vi "set FCC Part15c U-NII-1 Integration BE mode.vi"(8 "error in (no error)":errorcluster, 11 "Band Edge in":refnum<class "Band Edge.lvclass">) -> (0 "error out":errorcluster, 3 "Band Edge out":refnum<class "Band Edge.lvclass">)   [LabVIEW 2023, in "Spectrum Analyzer.lvlib" / "Band Edge.lvclass"]
uses:
  Band Edge.lvclass
  Band Edge.lvclass/Band Edge.ctl
  TYPE DEFINITION/TYPE RBW and VBW Select.ctl
  Spectrum Analyzer.lvlib
  TYPE DEFINITION/TYPE Reference Level and Atten Param.ctl
  TYPE DEFINITION/TYPE Y-axis Unit.ctl
  TYPE DEFINITION/TYPE Sweep Type Select.ctl
  Interface_Spectrum/Interface_Spectrum.lvclass
  TYPE DEFINITION/TYPE Measurement Window Mode.ctl
  TYPE DEFINITION/TYPE Average Mode Select.ctl
  TYPE DEFINITION/TYPE Marker Value.ctl
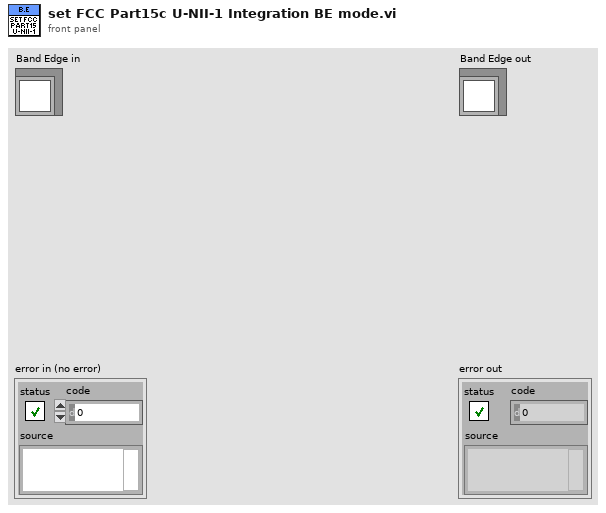
[diagram p1: front panel]
types:
  T1 = typedef "Spectrum Analyzer.lvlib/TYPE Marker Value.ctl" = cluster{"X-axis":dbl, "Y-axis":dbl}
  T2 = typedef "Spectrum Analyzer.lvlib/TYPE Measurement Window Mode.ctl" = enum16{"ACPower", "CPOWer", "MCACpower", "OBANdwidth", "OBWidth", "CN", "CN0"}
  T3 = typedef "Spectrum Analyzer.lvlib/TYPE Average Mode Select.ctl" = enum16{"Linear(Voltage Avg)", "Video(Log)", "Power"}
  T4 = typedef "Spectrum Analyzer.lvlib/TYPE Sweep Type Select.ctl" = enum16{"Auto", "Sweep", "FFT"}
  T5 = typedef "Spectrum Analyzer.lvlib/TYPE Y-axis Unit.ctl" = enum16{"dBm", "dBmV", "dBuV", "dBpW", "Volt", "Ampere", "Watt"}
  T6 = typedef "Spectrum Analyzer.lvlib/TYPE Reference Level and Atten Param.ctl" = cluster{"Reference Level":dbl, "Atten":i32, "Atten Auto?":bool, "Reference Level Offset":dbl}
  T7 = typedef "Spectrum Analyzer.lvlib/TYPE RBW and VBW Select.ctl" = enum16{"Res BW", "Video BW"}
  T8 = typedef "Spectrum Analyzer.lvlib/TYPE Spectrum Window Select.ctl" = enum16{"Spectrum 1", "Spectrum 2", "Spectrum 3", "Spectrum 4"}
  T9 = typedef "Spectrum Analyzer.lvlib/TYPE Start and Stop Frequency.ctl" = cluster{"Start":dbl, "Stop":dbl}
  T10 = typedef "Spectrum Analyzer.lvlib/TYPE Display Trace Mode Select.ctl" = enum16{"Clear Write", "Max Hold", "Min Hold", "Average", "View"}
  T11 = typedef "Spectrum Analyzer.lvlib/TYPE Detect Mode Select.ctl" = enum16{"Det Auto (Normal)", "Auto Peak", "Positive Peak", "Negative Peak", "Sample", "RMS", "Average", "Quasipeak", "CISPR Average", "RMS Average"}
  T12 = typedef "Spectrum Analyzer.lvlib/TYPE ACLR Setting Param.ctl" = cluster{"Bandwidth":dbl, "Offset":dbl, "Tx Channel Count":i32}
  T13 = typedef "Spectrum Analyzer.lvlib/TYPE Frequency Line Param.ctl" = cluster{"Line 1":dbl, "Line 2":dbl, "Activate Line1?":bool, "Activate Line2?":bool}
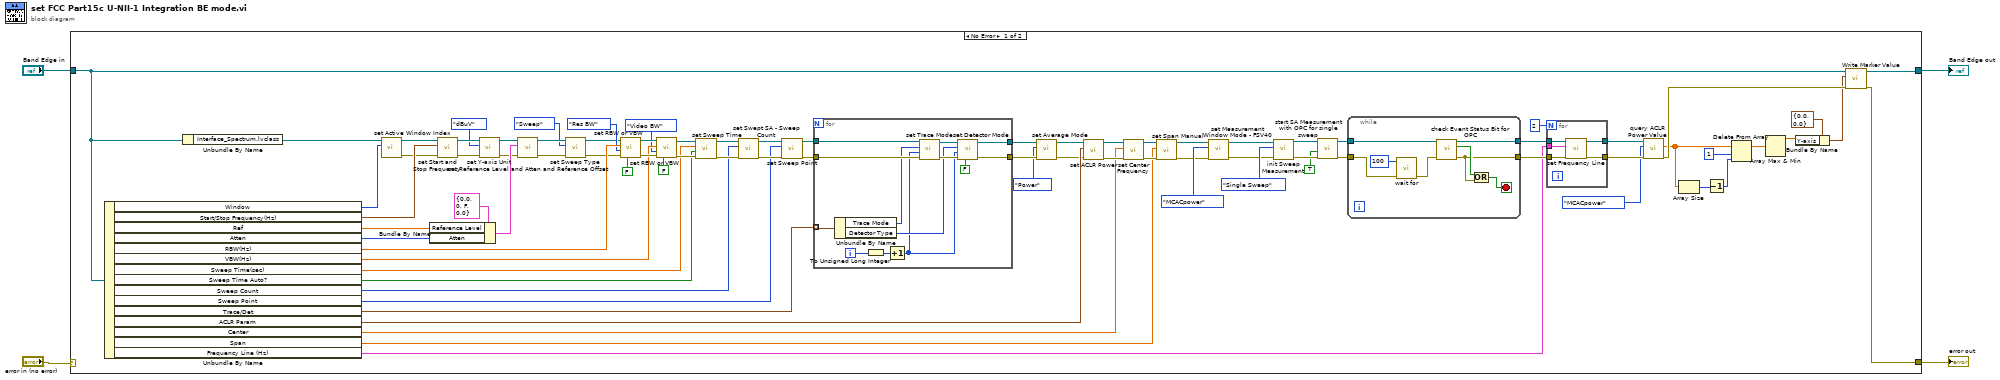
[diagram p0: block diagram]
diagram:
  n1 = case shown="No Error" "error in (no error)" {
    selector: "error in (no error)" -> [_ w114]
    tunnel: [w16 w114] -> w2
    tunnel: [w18 w113] -> w1
    tunnel: "Band Edge in" -> [w15 w113]
    frame No Error {
      n2 = Unbundle By Name(w15) -> ("Window"=w61:T8, "Start/Stop Frequency(Hz)"=w86:T9, "Ref"=w65:dbl, "Atten"=w64:i32, "RBW(Hz)"=w85:dbl, "VBW(Hz)"=w79:dbl, "Sweep Time(sec)"=w6:dbl, "Sweep Time Auto?"=w5:bool, "Sweep Count"=w73:u32, "Sweep Point"=w70:u32, "Trace/Det"=w67:cluster{"Trace Mode":T10, "Detector Type":T11}[], "ACLR Param"=w41:T12, "Center"=w38:dbl, "Span"=w35:dbl, "Frequency Line (Hz)"=w27:T13)
      n3 = Unbundle By Name(w15) -> ("Interface_Spectrum.lvclass"=w62:refnum<class "Interface_Spectrum.lvclass">)
      n4 = call-dynamic "set Active Window Index.vi"("Window"=w61, "Interface_Spectrum in"=w62) -> ("error out"=w59:errorcluster, "Interface_Spectrum out"=w60:refnum<class "Interface_Spectrum.lvclass">)  [unwired: 8 in]
      n5 = Bundle By Name(cluster=T6 {"Reference Level"=0.0, "Atten"=0, "Atten Auto?"=FALSE, "Reference Level Offset"=0.0} ("Ref and Atten"), "Reference Level"=w65, "Atten"=w64) -> (w63:T6)
      n6 = call-dynamic "set Start and Stop Frequency.vi"("error in (no error)"=w59, "Start/Stop Frequency(Hz)"=w86, "Interface_Spectrum in"=w60) -> ("error out"=w57:errorcluster, "Interface_Spectrum out"=w58:refnum<class "Interface_Spectrum.lvclass">)  [unwired: 7 in]
      n7 = call-dynamic "set Y-axis Unit.vi"("error in (no error)"=w57, "Y-axis Unit"=TYPE_Y-axis_Unit."dBuV", "Interface_Spectrum in"=w58) -> ("error out"=w55:errorcluster, "Interface_Spectrum out"=w56:refnum<class "Interface_Spectrum.lvclass">)  [unwired: 7 in]
      n8 = call-dynamic "set Reference Level and Atten and Reference Offset.vi"("error in (no error)"=w55, "Reference Level, Atten, Reference Offset"=w63, "Interface_Spectrum in"=w56) -> ("error out"=w52:errorcluster, "Interface_Spectrum out"=w53:refnum<class "Interface_Spectrum.lvclass">)  [unwired: 7 in]
      n9 = call-dynamic "set Sweep Type.vi"("error in (no error)"=w52, "Sweep Mode"=TYPE_Sweep_Type_Select."Sweep", "Interface_Spectrum in"=w53) -> ("error out"=w50:errorcluster, "Interface_Spectrum out"=w51:refnum<class "Interface_Spectrum.lvclass">)  [unwired: 7 in]
      n10 = call-dynamic "set RBW or VBW.vi"("BW Auto?"=FALSE, "error in (no error)"=w50, "BW Type"=TYPE_RBW_and_VBW_Select."Res BW", "BW Value (Hz)"=w85, "Interface_Spectrum in"=w51) -> ("error out"=w82:errorcluster, "Interface_Spectrum out"=w83:refnum<class "Interface_Spectrum.lvclass">)  [unwired: 5 in]
      n11 = call-dynamic "set RBW or VBW.vi"("BW Auto?"=FALSE, "error in (no error)"=w82, "BW Type"=TYPE_RBW_and_VBW_Select."Video BW", "BW Value (Hz)"=w79, "Interface_Spectrum in"=w83) -> ("error out"=w76:errorcluster, "Interface_Spectrum out"=w77:refnum<class "Interface_Spectrum.lvclass">)  [unwired: 5 in]
      n12 = call-dynamic "set Sweep Time.vi"("error in (no error)"=w76, "Sweep Time Auto?"=w5, "Sweep Time(sec)"=w6, "Interface_Spectrum in"=w77) -> ("error out"=w74:errorcluster, "Interface_Spectrum out"=w75:refnum<class "Interface_Spectrum.lvclass">)  [unwired: 6 in]
      n13 = call-dynamic "set Swept SA - Sweep Count.vi"("error in (no error)"=w74, "Sweep Count"=w73, "Interface_Spectrum in"=w75) -> ("error out"=w71:errorcluster, "Interface_Spectrum out"=w72:refnum<class "Interface_Spectrum.lvclass">)  [unwired: 7 in]
      n14 = call-dynamic "set Sweep Point.vi"("error in (no error)"=w71, "Sweep Point"=w70, "Interface_Spectrum in"=w72) -> ("error out"=w68:errorcluster, "Interface_Spectrum out"=w69:refnum<class "Interface_Spectrum.lvclass">)  [unwired: 7 in]
      n15 = for {
        tunnel: w69 -> [w112]
        tunnel: w68 -> [w111]
        tunnel: w67 -> [w107] mode=indexing
        tunnel: [w101] -> w26
        tunnel: [w100] -> w25
        i -> [w104]
        n16 = Unbundle By Name(w107) -> ("Trace Mode"=w106:T10, "Detector Type"=w105:T11)
        n17 = To Unsigned Long Integer(number=w104) -> (unsigned 32bit integer=w102:u32)
        n18 = Increment(x=w102) -> (x+1=w103:u32)
        n19 = call-dynamic "set Trace Mode.vi"("error in (no error)"=w111, "Trace Index"=w103, "Trace Mode"=w106, "Interface_Spectrum in"=w112) -> ("error out"=w109:errorcluster, "Interface_Spectrum out"=w110:refnum<class "Interface_Spectrum.lvclass">)  [unwired: 6 in]
        n20 = call-dynamic "set Detector Mode.vi"("Detect Auto?"=FALSE, "error in (no error)"=w109, "Trace Index"=w103, "Detector Type"=w105, "Interface_Spectrum in"=w110) -> ("error out"=w100:errorcluster, "Interface_Spectrum out"=w101:refnum<class "Interface_Spectrum.lvclass">)  [unwired: 5 in]
      }
      n21 = call-dynamic "set Average Mode.vi"("error in (no error)"=w25, "Average Mode"=TYPE_Average_Mode_Select."Power", "Interface_Spectrum in"=w26) -> ("error out"=w23:errorcluster, "Interface_Spectrum out"=w24:refnum<class "Interface_Spectrum.lvclass">)  [unwired: 7 in]
      n22 = call-dynamic "set ACLR Power.vi"("error in (no error)"=w23, "ACLR Param"=w41, "Interface_Spectrum in"=w24) -> ("error out"=w39:errorcluster, "Interface_Spectrum out"=w40:refnum<class "Interface_Spectrum.lvclass">)  [unwired: 7 in]
      n23 = call-dynamic "set Center Frequency.vi"("error in (no error)"=w39, "Center Frequency (Hz)"=w38, "Interface_Spectrum in"=w40) -> ("error out"=w36:errorcluster, "Interface_Spectrum out"=w37:refnum<class "Interface_Spectrum.lvclass">)  [unwired: 7 in]
      n24 = call-dynamic "set Span Manual.vi"("error in (no error)"=w36, "Span (Hz)"=w35, "Interface_Spectrum in"=w37) -> ("error out"=w30:errorcluster, "Interface_Spectrum out"=w31:refnum<class "Interface_Spectrum.lvclass">)  [unwired: 7 in]
      n25 = call-dynamic "set Measurement Window Mode - FSV40.vi"("error in (no error)"=w30, "Measurement Window Mode"=TYPE_Measurement_Window_Mode."MCACpower", "Interface_Spectrum in"=w31) -> ("error out"=w32:errorcluster, "Interface_Spectrum out"=w33:refnum<class "Interface_Spectrum.lvclass">)  [unwired: 7 in]
      n26 = call-dynamic "init Sweep Measurement.vi"("error in (no error)"=w32, "Sweep Measurement Mode"=enum16{"Single Sweep", "Continuous Sweep"}."Single Sweep", "Interface_Spectrum in"=w33) -> ("error out"=w45:errorcluster, "Interface_Spectrum out"=w46:refnum<class "Interface_Spectrum.lvclass">)  [unwired: 7 in]
      n27 = call-dynamic "start SA Measurement with OPC for single sweep.vi"("error in (no error)"=w45, "with OPC?"=TRUE ("Check OPC?"), "Interface_Spectrum in"=w46) -> ("error out"=w42:errorcluster, "Interface_Spectrum out"=w43:refnum<class "Interface_Spectrum.lvclass">)  [unwired: 7 in]
      n28 = while {
        tunnel: w43 -> [w94]
        tunnel: w42 -> [w93]
        tunnel: [w89] -> w28
        tunnel: [w87] -> w29
        stop <- w90 stop-if-true
        n29 = call "wait for.vi"("error in"=w93, "Wait Time (ms)"=100) -> ("error out"=w92:errorcluster)  [unwired: 9 in]
        n30 = call-dynamic "check Event Status Bit for OPC.vi"("error in (no error)"=w92, "Interface_Spectrum in"=w94) -> ("error out"=w89:errorcluster, "OPC Bit Changed?"=w91:bool, "Interface_Spectrum out"=w87:refnum<class "Interface_Spectrum.lvclass">)  [unwired: 7 in]
        n31 = Or(x=w91, y=w89) -> (x .or. y?=w90:bool)
      }
      n32 = for {
        N: 2 -> [_]
        tunnel: w29 -> [w99]
        tunnel: w28 -> [w98]
        tunnel: w27 -> [w97]
        tunnel: [w96] -> w21
        tunnel: [w95] -> w20
        n33 = call-dynamic "set Frequency Line.vi"("error in (no error)"=w98, "Frequency Line (Hz)"=w97, "Interface_Spectrum in"=w99) -> ("error out"=w95:errorcluster, "Interface_Spectrum out"=w96:refnum<class "Interface_Spectrum.lvclass">)  [unwired: 7 in]
      }
      n34 = call-dynamic "query ACLR Power Value.vi"("error in (no error)"=w20, "Measurement Window Mode"=TYPE_Measurement_Window_Mode."MCACpower", "Interface_Spectrum in"=w21) -> ("error out"=w17:errorcluster, "Channel Powers"=w10:dbl[])  [unwired: 6 in, 1 out]
      n35 = Array Size(array=w10) -> (size(s)=w8:i32)
      n36 = Decrement(x=w8) -> (x-1=w7:i32)
      n37 = Delete From Array(array=w10, length=1, index=w7) -> (array with subset deleted=w11:dbl[])  [unwired: 1 out]
      n38 = Array Max & Min(array=w11) -> (max value=w13:dbl)  [unwired: 3 out]
      n39 = Bundle By Name(cluster=T1 {"X-axis"=0.0, "Y-axis"=0.0} ("Marker Value"), "Y-axis"=w13) -> (w12:T1)
      n40 = call "Write Marker Value.vi"("error in (no error)"=w17, "Marker Value"=w12, "Band Edge in"=w15) -> ("error out"=w16:errorcluster, "Band Edge out"=w18:refnum<class "Band Edge.lvclass">)  [unwired: 7 in]
    }
    frame Error {
    }
  }
  "error out" <- w2
  "Band Edge out" <- w1
